vi "UNITTEST-JSON-RPC-typedef-cluster.vi"(8 "error in (no error)":errorcluster) -> (0 "error out":errorcluster)   [LabVIEW 2019]
uses:
  TEST-JSON-RPC--Cluster.ctl
  <vilib>/numeric/Random Number (Range) DBL.vi
  4c12f335-3af6-49f5-9257-0130b4f6318c.vi
  e861ad0b-bed5-4796-b07d-8449c8f87c08.vi
  JSON-RPC/API/JSON to Variant.vi
  <vilib>/Utility/Data Type/Get Type Information.vi
  <vilib>/JDP Science/JSONtext/JSON type.vi
  <vilib>/JDP Science/JSONtext/Get Array Elements.vi
  <vilib>/JDP Science/JSONtext/JSON text to Variant.vi
  <vilib>/addons/_JKI Toolkits/Caraya/classes/Assert/Assert Almost Equal_Float.vi
  <vilib>/addons/_JKI Toolkits/Caraya/classes/Assert/Assert Not Error.vi
  JSON-RPC/JSON-RPC.lvlib
  <vilib>/addons/_JKI Toolkits/Caraya/classes/Assert/Assert.lvclass
  <vilib>/addons/_JKI Toolkits/Caraya/classes/Test/Test.lvclass
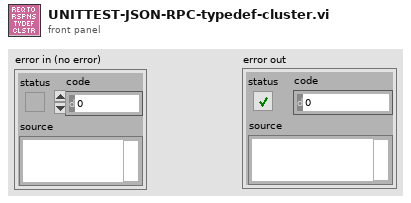
[diagram p1: front panel]
types:
  T1 = typedef "TEST-JSON-RPC--Cluster.ctl" = cluster{"Temperature (K)":dbl, "Rate (K/min)":dbl}
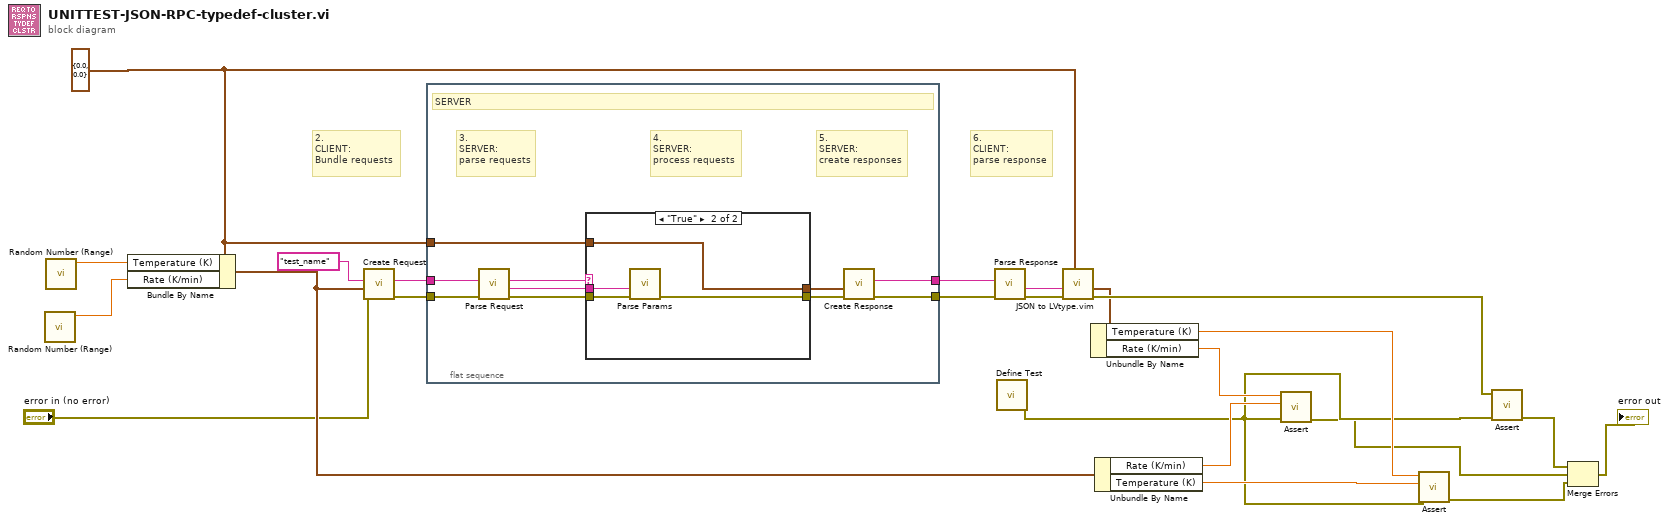
[diagram p0: block diagram]
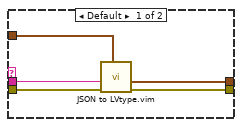
[diagram p2: hidden frame]
diagram:
  w6 = T1 {"Temperature (K)"=0.0, "Rate (K/min)"=0.0} ("Cluster")
  # "6.\nCLIENT:\nparse response"
  # "2.\nCLIENT:\nBundle requests"
  n1 = call-poly <vilib>:"Random Number (Range).vi"() -> ("number"=w19:dbl)  [unwired: 11 in]
  n2 = call-poly <vilib>:"Random Number (Range).vi"() -> ("number"=w18:dbl)  [unwired: 11 in]
  n3 = Bundle By Name(cluster=w6, "Temperature (K)"=w18, "Rate (K/min)"=w19) -> (w10:T1)
  n4 = call "Create Request.vi"("error in (no error)"="error in (no error)", "params"=w10, "method"="test_name") -> ("error out"=w22:errorcluster, "<JSON> Requests"=w23:string)  [unwired: 6 in, 1 out]
  n5 = flat-sequence {
    tunnel: w23 -> [w33]
    tunnel: w22 -> [w29]
    tunnel: [w28] -> w21
    tunnel: [w27] -> w20
    tunnel: w6 -> [w25]
    frame #0 {
      # "3.\nSERVER:\nparse requests"
      # "4.\nSERVER:\nprocess requests"
      # "5.\nSERVER:\ncreate responses"
      # "SERVER"
      n6 = call "Parse Request.vi"("error in (no error)"=w29, "<JSON> Requests"=w33) -> ("error out"=w30:errorcluster, "Params"=w31:string, "Methods"=w32:string)  [unwired: 6 in, 1 out]
      n7 = case shown="\"True\"" w32 {
        tunnel: w31 -> [w35 w42]
        tunnel: w30 -> [w38 w41]
        tunnel: [w37 w40] -> w26
        tunnel: w25 -> [w36 w39]
        tunnel: [w34 w39] -> w24
        frame Default {
          n8 = call "JSON to LVtype.vim"("type"=w36, "error in (no error)"=w38, "JSON Data in"=w35) -> ("error out"=w37:errorcluster, "Data out"=w34:T1)  [unwired: 7 in]
        }
        frame "True" {
          n9 = call "Parse Params.vi"("error in (no error)"=w41, "<JSON> Params"=w42) -> ("error out"=w40:errorcluster)  [unwired: 7 in, 2 out]
        }
      }
      n10 = call "Create Response.vi"("error in (no error)"=w26, "result"=w24) -> ("error out"=w27:errorcluster, "<JSON> Response"=w28:string)  [unwired: 8 in]
    }
  }
  n11 = call "Parse Response.vi"("error in (no error)"=w20, "<JSON> Response"=w21) -> ("error out"=w17:errorcluster, "results"=w8:string)  [unwired: 7 in, 1 out]
  n12 = call <vilib>:"Define Test.vi"() -> ("error out"=w2:errorcluster)  [unwired: 10 in, 1 out]
  n13 = call "JSON to LVtype.vim"("type"=w6, "error in (no error)"=w17, "JSON Data in"=w8) -> ("error out"=w12:errorcluster, "Data out"=w7:T1)  [unwired: 7 in]
  n14 = Unbundle By Name(w7) -> ("Temperature (K)"=w15:dbl, "Rate (K/min)"=w16:dbl)
  n15 = Unbundle By Name(w10) -> ("Rate (K/min)"=w14:dbl, "Temperature (K)"=w13:dbl)
  n16 = call-poly <vilib>:"Assert.vi"("error in (no error)"=w2, "Actual"=w14, "Expected"=w16) -> ("error out"=w1:errorcluster)  [unwired: 7 in, 1 out]
  n17 = call-poly <vilib>:"Assert.vi"("error in (no error)"=w2, "Actual"=w13, "Expected"=w15) -> ("error out"=w5:errorcluster)  [unwired: 7 in, 1 out]
  n18 = call-poly <vilib>:"Assert.vi"("error in (no error)"=w2, "Not Error?"=w12) -> ("error out"=w4:errorcluster)  [unwired: 8 in, 1 out]
  n19 = Merge Errors(w4, w1, w5) -> (→"error out":errorcluster)
